vi "Task List.vi"(7 "Project Store in":refnum<class "Project Store.lvclass">, 8 "error in":errorcluster, 11 "Project ID":string) -> (0 "error out":errorcluster, 2 "Task IDs":string[](array[string]), 3 "Task Names":string[](array[string]), 5 "Project Store out":refnum<class "Project Store.lvclass">)   [LabVIEW 2026]
doc: "Returns the active tasks of one project in Sort Order, as the parallel arrays a ring or listbox needs: Task Names for display and Task IDs to look up the selection. Inactive tasks are left out. An empty or unknown Project ID gives two empty arrays and no error. Tasks are matched by Project ID, so the same task name in two projects gives two different IDs.\n\nInputs: Project ID; Project Store in (already read from its data source); error in.\nOutputs: Task Names; Task IDs (same order as Task Names); Project Store out; error out.\n\nGenerated by: Claude"
uses:
  Storage/Project Store/Project Store.lvclass
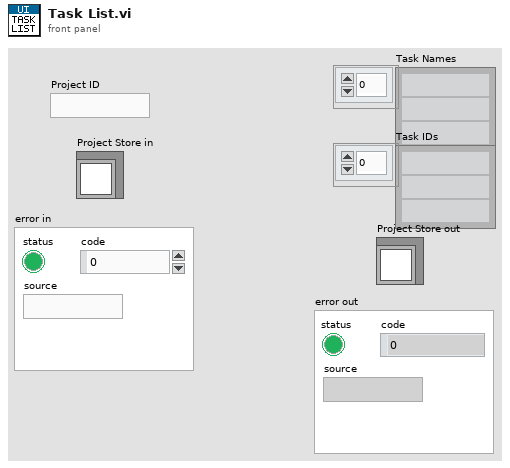
[diagram p1: front panel]
types:
  T1 = typedef "Task List.ctl" = T2[]
  T2 = typedef "Task.ctl" = cluster{"ID":string, "Project ID":string, "Name":string, "Active":bool, "Sort Order":i32}
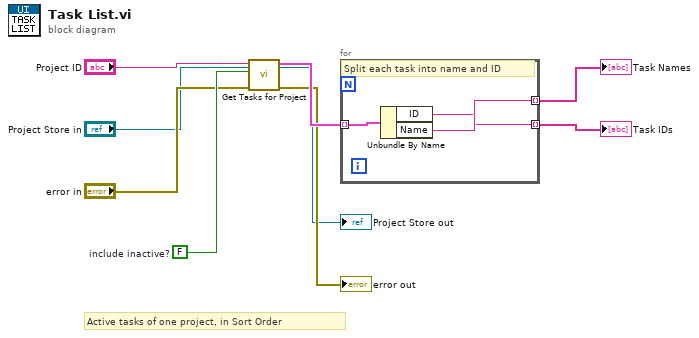
[diagram p0: block diagram]
diagram:
  w8 = FALSE  # include inactive?
  # "Active tasks of one project, in Sort Order"
  n1 = call-dynamic "Get Tasks for Project.vi"("Project Store in"="Project Store in", "error in (no error)"="error in", "include inactive?"=w8, "Project ID"="Project ID") -> ("error out"=→"error out":errorcluster, "Tasks"=w9:T1, "Project Store out"=→"Project Store out":refnum<class "Project Store.lvclass">)  [unwired: 5 in]
  n2 = for {
    tunnel: w9 -> [w10] mode=indexing
    tunnel: [w12] -> w4 mode=indexing
    tunnel: [w11] -> w5 mode=indexing
    # "Split each task into name and ID"
    n3 = Unbundle By Name(w10) -> ("ID"=w11:string, "Name"=w12:string)
  }
  "Task Names" <- w4
  "Task IDs" <- w5
